vi "CSE routine - Runtime Link Scripts Core.vi"(6 "action":i32(ring) items=["save vi path", "link to caller", "delink of caller", "call-chain info"], 7 "Caller CSE RefNum":T1, 8 "error in":errorcluster, 10 "Callback VI Path":path, 11 "CSE RefNum":T1) -> (0 "error out":errorcluster, 1 "Script Name":string, 2 "Callback VI Path out":path, 3 "dup CSE RefNum":T1, 4 "Caller Run mode":T3 items=["Execute", "Abort", "Run", "Step", "Step Over", "Step Out", "Run (LM)", "Step (LM)", "Step Over (LM)", "Step Out (LM)", "unsupported"], 5 "call-chain info":T2)   [LabVIEW 2021]
doc: "::: CalcExpress Toolkit :::\nCopyright (c) 2000-2026 Konstantin Shifershteyn. All rights reserved."
uses:
  CSE Instance RefNum.ctl
  CSE Type - Run Mode.ctl
  cersrc/celveng32.dll
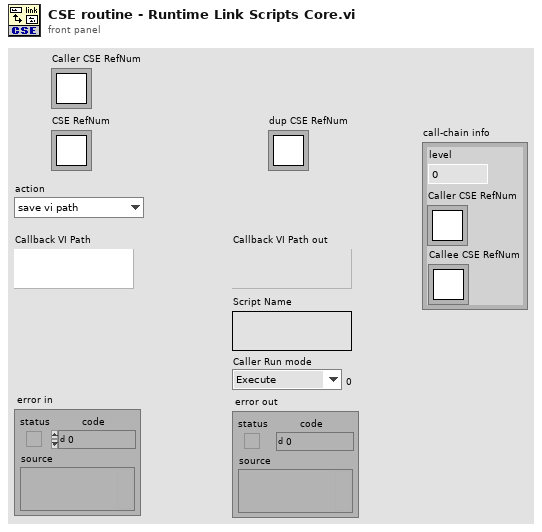
[diagram p1: front panel]
types:
  T1 = typedef "CSE Instance RefNum.ctl" = refnum<k1>
  T2 = cluster{"level":i32, "Caller CSE RefNum":T1, "Callee CSE RefNum":T1}
  T3 = typedef "CSE Type - Run Mode.ctl" = u32
  T4 = cluster{i32, "Caller CSE RefNum":T1, "Caller CSE RefNum":T1}
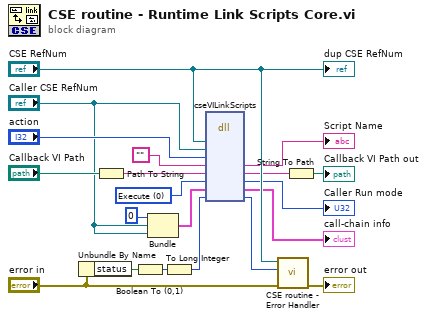
[diagram p0: block diagram]
diagram:
  w11 = T3 0 items=["Execute", "Abort", "Run", "Step", "Step Over", "Step Out", "Run (LM)", "Step (LM)", "Step Over (LM)", "Step Out (LM)", "unsupported"] ("Run mode")
  n1 = Unbundle By Name("error in") -> ("status"=w17:bool)
  n2 = Path To String(path="Callback VI Path") -> (string=w12:string)
  n3 = Boolean To (0,1)(Boolean=w17) -> (0, 1=w18:i16)
  n4 = Bundle(0, "Caller CSE RefNum"="Caller CSE RefNum", "Caller CSE RefNum"="Caller CSE RefNum") -> (w2:T4)  [unwired: 1 in]
  n5 = To Long Integer(number=w18) -> (32bit integer=w6:i32)
  n6 = dll-call lib="C:/LV Projects/CalcExpress 40 LV2021/vi.lib/addons/CalcExpress/cersrc/celveng*.dll" fn="cseVILinkScripts"("iRef"="CSE RefNum", "iRefCaller"="Caller CSE RefNum", "cmd"="action", "srciptName"="", "cbPath"=w12, "runMode"=w11, "ccInfo"=w2, "erStat"=w6) -> ("srciptName"=→"Script Name":string, "cbPath"=w10:string, "runMode"=→"Caller Run mode":T3, "ccInfo"=→"call-chain info":T4, "erStat"=w5:i32)  [unwired: 7 in, 2 out]
  n7 = call "CSE routine - Error Handler.vi"("error in"="error in", "exec status"=w5, "CSE RefNum"="CSE RefNum") -> ("error out"=→"error out":errorcluster)  [unwired: 4 in, 2 out]
  n8 = String To Path(string=w10) -> (path=→"Callback VI Path out":path)
  "dup CSE RefNum" <- "CSE RefNum"
